vi "ZM-CI-handlePackage.vi"(8 "error in (no error)":errorcluster, 10 "package":refnum<class "ZM-PC-package.lvclass">, 11 "ZM-HWM-hardware_manager in":refnum<class "ZM-HWM-hardware_manager.lvclass">) -> (0 "error out":errorcluster, 3 "ZM-HWM-hardware_manager out":refnum<class "ZM-HWM-hardware_manager.lvclass">)   [LabVIEW 2020, in "ZM-HWM-hardware_manager.lvlib" / "ZM-HWM-hardware_manager.lvclass"]
doc: "The hardware manager's ZM-CI-handlePackage override, called for each package its helper loop sends: counts the package and forwards it to its caller (the root). A failed send (the caller already gone at shutdown) is cleared."
uses:
  ZM-HWM-hardware_manager.lvclass
  common/ZM-PC-packages/ZM-PC-package/ZM-PC-package.lvclass
  ZM-HWM-hardware_manager.lvclass/ZM-HWM-hardware_manager.ctl
  common/ZM-CI-common_interfaces/ZM-CI-handlePackage Msg/ZM-CI-handlePackage Msg.lvclass
  <vilib>/ActorFramework/Actor/Actor.lvclass
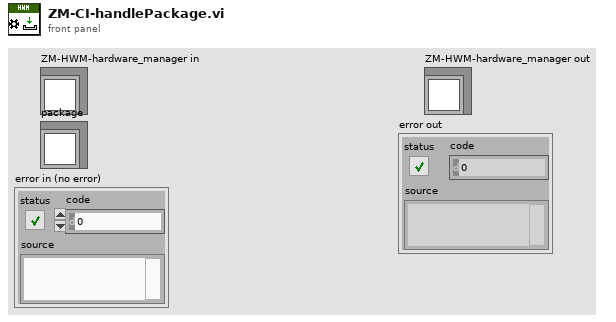
[diagram p1: front panel]
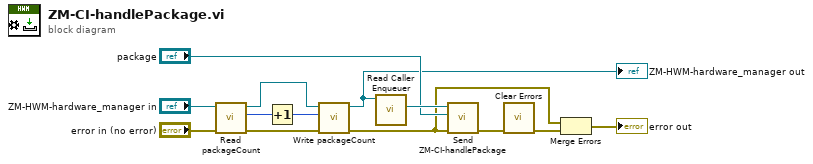
[diagram p0: block diagram]
diagram:
  n1 = call "Read packageCount.vi"("error in (no error)"="error in (no error)", "ZM-HWM-hardware_manager in"="ZM-HWM-hardware_manager in") -> ("error out"=w10:errorcluster, "packageCount"=w11:u32, "ZM-HWM-hardware_manager out"=w9:refnum<class "ZM-HWM-hardware_manager.lvclass">)  [unwired: 7 in]
  n2 = Increment(x=w11) -> (x+1=w8:u32)
  n3 = call "Write packageCount.vi"("error in (no error)"=w10, "packageCount"=w8, "ZM-HWM-hardware_manager in"=w9) -> ("error out"=w4:errorcluster, "ZM-HWM-hardware_manager out"=w2:refnum<class "ZM-HWM-hardware_manager.lvclass">)  [unwired: 7 in]
  "ZM-HWM-hardware_manager out" <- w2
  n4 = call <vilib>:"Read Caller Enqueuer.vi"("Actor"=w2) -> ("Caller Enqueuer"=w7:refnum<class "Message Enqueuer.lvclass">)  [unwired: 10 in]
  n5 = call "Send ZM-CI-handlePackage.vi"("error in (no error)"=w4, "package"="package", "Message Enqueuer"=w7) -> ("error out"=w5:errorcluster)  [unwired: 7 in, 1 out]
  n6 = call <vilib>:"Clear Errors.vi"("error in (no error)"=w5) -> ("error out"=w3:errorcluster)  [unwired: 5 in, 1 out]
  n7 = Merge Errors(w4, w3) -> (→"error out":errorcluster)
